vi "DAQ.Simulate Noisy AI.vi"(6 "Waveguide Cluster":T1={"I+"=0, "I-"=1, "V+"=2, "V-"=3, "Vsg"=4}, 8 "error in (no error)":errorcluster, 11 "Instrument.DAQ in":refnum<class "Instrument.DAQ.lvclass">) -> (0 "error out":errorcluster, 2 "Noisy Signal Graph":waveform(dbl)[](graph), 3 "Instrument.DAQ out":refnum<class "Instrument.DAQ.lvclass">, 4 "AI time (s)":dbl format="%#_6p")   [LabVIEW 2019, in "Instrument.Lockin.lvlib" / "Instrument.DAQ.lvclass"]
uses:
  Instrument.DAQ.lvclass
  Simulate/Waveguide Model--Cluster.ctl
  Instrument.DAQ.lvclass/Instrument.DAQ.ctl
panel:
  out "Signal Graph":waveform(dbl)[](graph)
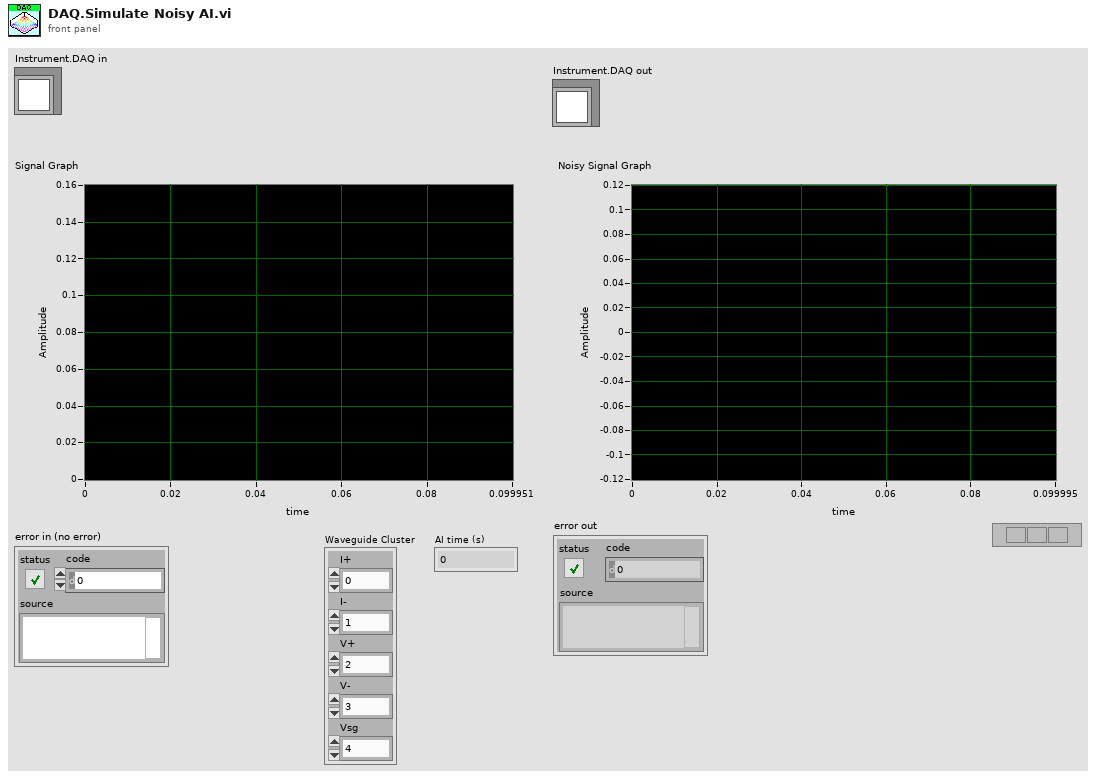
[diagram p1: front panel]
types:
  T1 = typedef "Instrument.Lockin.lvlib/Instrument.DAQ.lvclass/Waveguide Model--Cluster.ctl" = cluster{"I+":i32, "I-":i32, "V+":i32, "V-":i32, "Vsg":i32}
  T2 = typedef "Instrument.Lockin.lvlib/Instrument.DAQ.lvclass/Simulation Mode--enum.ctl" = enum16{"AI = HW simulated", "AI = noise*AO", "AI = waveguide"}
  T3 = typedef "Instrument.Lockin.lvlib/Instrument.DAQ.lvclass/DAQ.Sampling.Sampling--Cluster.ctl" = cluster{"Fs":dbl, "#s":i32}
  T4 = typedef "Instrument.Lockin.lvlib/Instrument.DAQ.lvclass/DeviceInfo--Cluster.ctl" = cluster{"DeviceName":string, "DevIsSimulated":bool, "DeviceSerialNumber":string, "ProductType":string, "ProductCategory":i32, "ProductNumber":u32, "ChassisNumber":u32, "SlotNumber":u32, "ChassisName":string, "ChassisSerialNumber":string, "DevTemp":dbl, "SelfCal.LastDate/Time":string, "SelfCal.LastTemp":dbl, "calibration due?":bool}
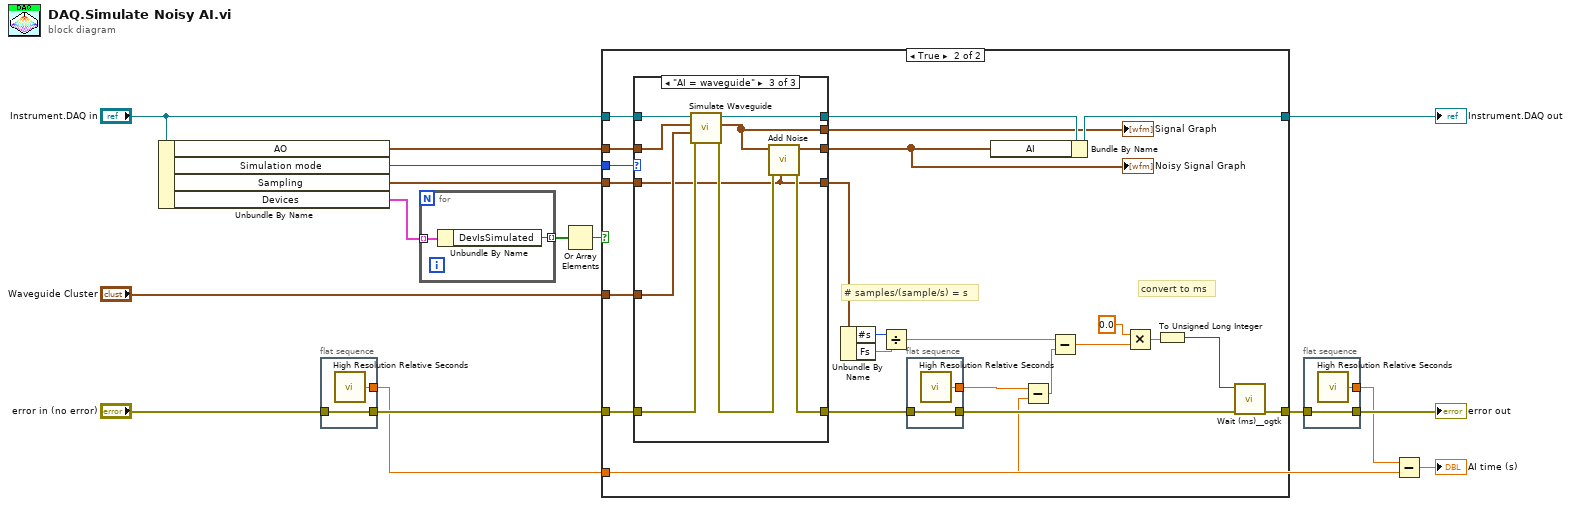
[diagram p0: block diagram]
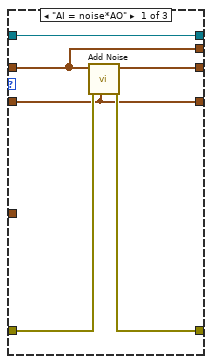
[diagram p3: hidden frame]
diagram:
  n1 = Unbundle By Name("Instrument.DAQ in") -> ("AO"=w15:waveform(dbl)[], "Simulation mode"=w14:T2, "Sampling"=w4:T3, "Devices"=w1:T4[])
  n2 = flat-sequence {
    tunnel: [w18] -> w10
    tunnel: "error in (no error)" -> [w18]
    tunnel: [w17] -> w6
    frame #0 {
      n3 = call <vilib>:"High Resolution Relative Seconds.vi"() -> ("relative seconds"=w17:dbl)
    }
  }
  n4 = for {
    tunnel: w1 -> [w20] mode=indexing
    tunnel: [w19] -> w3 mode=indexing
    n5 = Unbundle By Name(w20) -> ("DevIsSimulated"=w19:bool)
  }
  n6 = Or Array Elements(Boolean array=w3) -> (logical OR=w2:bool)
  n7 = case shown="True" w2 {
    tunnel: "Waveguide Cluster" -> [_ w43]
    tunnel: w15 -> [_ w41]
    tunnel: w14 -> [_ w40]
    tunnel: "Instrument.DAQ in" -> [w22 w39]
    tunnel: [w22 w38] -> w12
    tunnel: w10 -> [w21 w36]
    tunnel: [w21 w28] -> w9
    tunnel: w6 -> [_ w27]
    tunnel: w4 -> [_ w26]
    frame False {
    }
    frame True {
      # "convert to ms"
      # "# samples/(sample/s) = s"
      n8 = case shown="\"AI = waveguide\"" w40 {
        tunnel: w36 -> [w51 w57 w65]
        tunnel: [w52 w57 w61] -> w42
        tunnel: [w53 w55 w63] -> w23
        tunnel: w43 -> [_ _ w64]
        tunnel: w41 -> [w49 w55 w68]
        tunnel: w39 -> [w54 w58 w67]
        tunnel: [w54 w58 w66] -> w37
        tunnel: w26 -> [w50 w56 w60]
        tunnel: [w50 w56 w60] -> w25
        tunnel: [w49 w55 w59] -> w24
        frame "AI = noise*AO" {
          n9 = call "Add Noise.vi"("Sampling"=w50, "error in (no error)"=w51, "AI []"=w49) -> ("error out"=w52:errorcluster, "AI + Noise"=w53:waveform(dbl)[])  [unwired: 7 in]
        }
        frame "AI = HW simulated" {
        }
        frame "AI = waveguide" {
          n10 = call "Simulate Waveguide.vi"("error in (no error)"=w65, "Waveguide Cluster"=w64, "AO"=w68, "Instrument.DAQ in"=w67) -> ("error out"=w62:errorcluster, "AI"=w59:waveform(dbl)[], "Instrument.DAQ out"=w66:refnum<class "Instrument.DAQ.lvclass">)  [unwired: 5 in]
          n11 = call "Add Noise.vi"("Sampling"=w60, "error in (no error)"=w62, "AI []"=w59) -> ("error out"=w61:errorcluster, "AI + Noise"=w63:waveform(dbl)[])  [unwired: 7 in]
        }
      }
      "Noisy Signal Graph" <- w23
      "Signal Graph" <- w24
      n12 = Unbundle By Name(w25) -> ("#s"=w44:i32, "Fs"=w45:dbl)
      n13 = Divide(x=w44, y=w45) -> (x/y=w33:dbl)
      n14 = flat-sequence {
        tunnel: [w48] -> w35
        tunnel: w42 -> [w48]
        tunnel: [w47] -> w34
        frame #0 {
          n15 = call <vilib>:"High Resolution Relative Seconds.vi"() -> ("relative seconds"=w47:dbl)
        }
      }
      n16 = Bundle By Name(cluster=w37, "AI"=w23) -> (w38:refnum<class "Instrument.DAQ.lvclass">)
      n17 = Subtract(x=w34, y=w27) -> (x-y=w46:dbl)
      n18 = Subtract(x=w33, y=w46) -> (x-y=w30:dbl)
      n19 = Multiply(x=0.0, y=w30) -> (x*y=w32:dbl)
      n20 = To Unsigned Long Integer(number=w32) -> (unsigned 32bit integer=w29:u32)
      n21 = call <userlib>:"Wait (ms)__ogtk.vi"("error in (no error)"=w35, "milliseconds to wait"=w29) -> ("error out"=w28:errorcluster)  [unwired: 8 in, 1 out]
    }
  }
  "Instrument.DAQ out" <- w12
  n22 = flat-sequence {
    tunnel: [w70] -> w8
    tunnel: w9 -> [w70]
    tunnel: [w69] -> w7
    frame #0 {
      n23 = call <vilib>:"High Resolution Relative Seconds.vi"() -> ("relative seconds"=w69:dbl)
    }
  }
  n24 = Subtract(x=w7, y=w6) -> (x-y=→"AI time (s)":dbl)
  "error out" <- w8
